vi "InitLinkButtons.vi"(4 "Separator":refnum<vi>, 5 "rightColumnAlignment":refnum<vi>, 6 "Col1Sec3_Top":refnum<vi>, 7 "leftColumnAlignment":refnum<vi>, 8 "icon array":refnum<vi>[](array[refnum]), 9 "button array":refnum<vi>[][](array[refnum]), 10 "Num MRU Items":u16=10, 11 "Pnl Refnum":refnum<vi>) -> (0 "Mode XML Elements":string, 1 "ring info":refnum<class "RingItem.lvclass">[](array[class]), 3 "Handler info":variant)   [LabVIEW 2023, in "GettingStartedWindow.lvlib"]
uses:
  <resource>/modes/FRC/GSW/GettingStartedWindow.lvlib
  <resource>/modes/FRC/GSW/Classes/RingItem/RingItem.lvclass
  <resource>/modes/FRC/GSW/Classes/ClickableText/ClickableText.lvclass
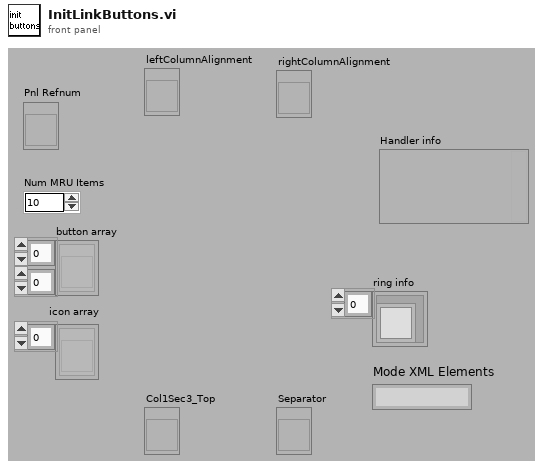
[diagram p1: front panel]
types:
  T1 = cluster{refnum<class "ClickableText.lvclass">[]}[][]
  T2 = typedef "GettingStartedWindow.lvlib/ItemData_Type.ctl" = enum16{"None", "Folder", "New Project", "New VI", "Find", "VI", "Project", "New from template", "RT Project Wizard", "PDA Project Wizard", "Control", "Library", "Class", "XControl", "Runtime menu", "Statechart", "Ladder", "Find LabVIEW Addons", "Instrument Finder", "Example Finder"}
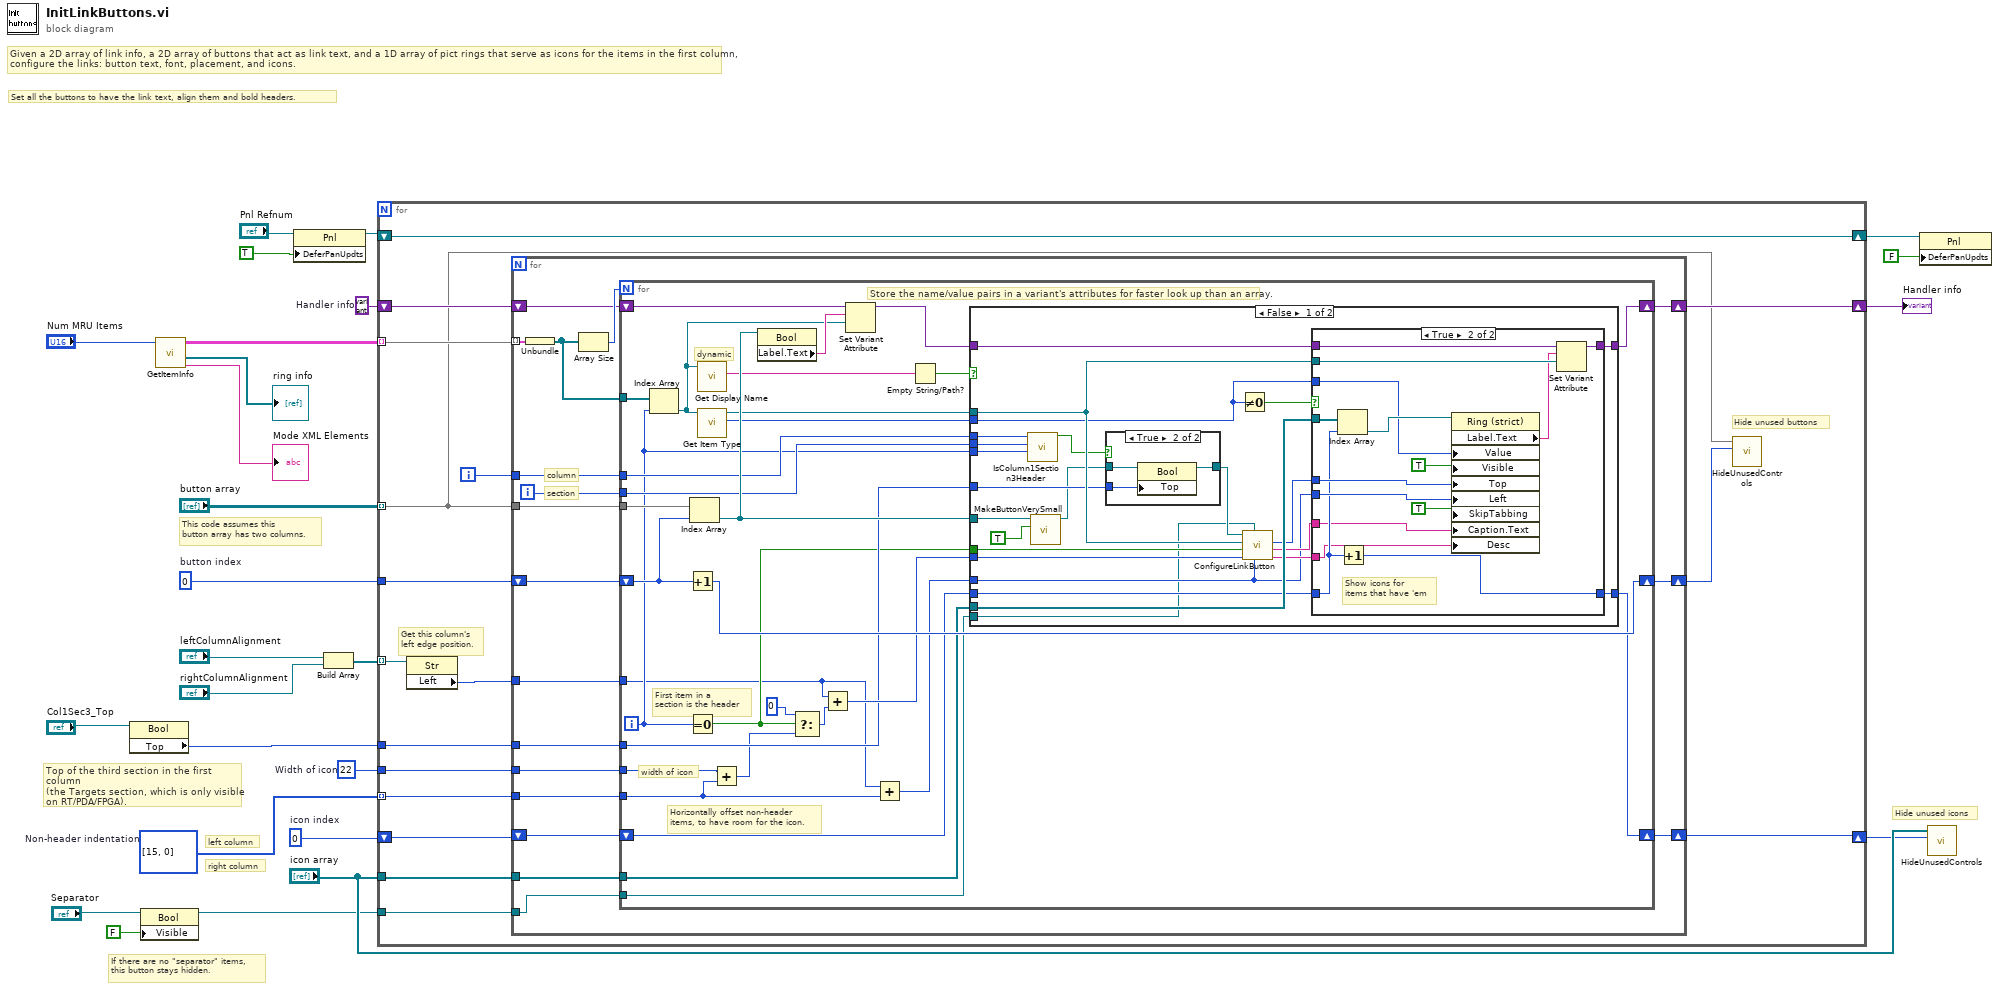
[diagram p0: block diagram]
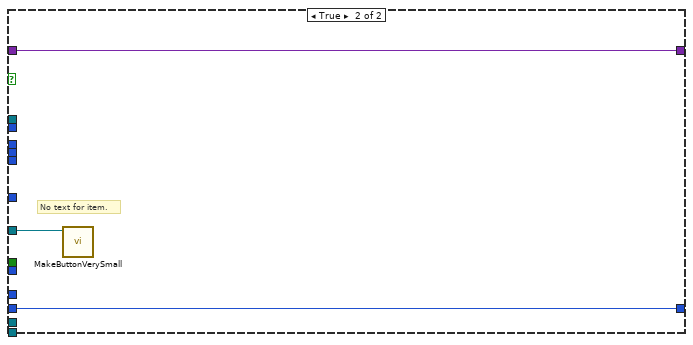
[diagram p4: hidden frame]
diagram:
  w5 = i32[] [15, 0]  # Non-header indentation
  w6 = 0  # button index
  w8 = variant  # Handler info
  w15 = 22  # Width of icon
  w19 = 0  # icon index
  # "If there are no \"separator\" items,\nthis button stays hidden."
  # "right column"
  # "left column"
  # "Set all the buttons to have the link text, align them and bold headers."
  # "Top of the third section in the first column\n(the Targets section, which is only visible\non RT/PDA/FPGA)."
  # "Given a 2D array of link info, a 2D array of buttons that act as link text, and a 1D array of pict rings that serve as icons for the items in the first column,\nconfigure the links: button text, font, placement, and icons."
  # "This code assumes this\nbutton array has two columns."
  # "Hide unused icons"
  n1 = property on="Property Node" class="Bool"(reference="Col1Sec3_Top") -> ("Top"=w12:i32)  [unwired: 1 in, 2 out]
  n2 = property class="Bool"(reference="Separator", "Visible"=FALSE) -> (reference out=w2:refnum<vi>)  [unwired: 1 in, 1 out]
  n3 = call <resource>:"GetItemInfo.vi"("Num MRU Items"="Num MRU Items") -> ("Mode XML Elements"=→"Mode XML Elements":string, "ring info"=→"ring info":refnum<class "RingItem.lvclass">[], "item info array"=w25:T1)  [unwired: 1 in, 7 out]
  n4 = property on="Property Node" class="Pnl"(reference="Pnl Refnum", "DeferPanUpdts"=TRUE ("Defer Panel Updates")) -> (reference out=w22:refnum<vi>)  [unwired: 1 in, 1 out]
  n5 = Build Array("leftColumnAlignment", "rightColumnAlignment") -> (w16:refnum<vi>[])
  n6 = for {
    tunnel: "button array" -> [w31] mode=indexing
    tunnel: w25 -> [w42] mode=indexing
    tunnel: "icon array" -> [w41]
    shift-right: [w39] -> w7
    shift-left: w8 -> [w40]
    shift-right: [w38] -> w20
    shift-left: w22 -> [w38]
    tunnel: w15 -> [w37]
    shift-right: [w35] -> w10
    shift-left: w19 -> [w36]
    tunnel: w16 -> [w34] mode=indexing
    tunnel: w12 -> [w33]
    tunnel: w6 -> [w29]
    tunnel: w5 -> [w28] mode=indexing
    tunnel: w2 -> [w27]
    i -> [w32]
    # "Get this column's\nleft edge position."
    # "Hide unused buttons"
    n7 = property on="Property Node" class="Str"(reference=w34) -> ("Left"=w43:i32)  [unwired: 1 in, 2 out]
    n8 = for {
      tunnel: w31 -> [w61]
      tunnel: w42 -> [w50] mode=indexing
      shift-right: [w59] -> w30
      shift-left: w29 -> [w60]
      tunnel: w43 -> [w58]
      shift-right: [w46] -> w39
      shift-left: w40 -> [w47]
      shift-right: [w56] -> w35
      shift-left: w36 -> [w57]
      tunnel: w41 -> [w55]
      tunnel: w37 -> [w54]
      tunnel: w33 -> [w53]
      tunnel: w32 -> [w52]
      tunnel: w28 -> [w45]
      tunnel: w27 -> [w44]
      i -> [w51]
      # "section"
      # "column"
      n9 = Unbundle(w50) -> (w48:refnum<class "ClickableText.lvclass">[])
      n10 = Array Size(array=w48) -> (size(s)=w49:i32)
      n11 = for {
        N: w49 -> [_]
        tunnel: w48 -> [w86]
        tunnel: w61 -> [w92]
        shift-right: [w90] -> w59
        shift-left: w60 -> [w91]
        tunnel: w58 -> [w65]
        shift-right: [w83] -> w56
        shift-left: w57 -> [w84]
        tunnel: w55 -> [w73]
        tunnel: w54 -> [w67]
        tunnel: w53 -> [w82]
        tunnel: w52 -> [w81]
        tunnel: w51 -> [w80]
        shift-right: [w69] -> w46
        shift-left: w47 -> [w74]
        tunnel: w45 -> [w64]
        tunnel: w44 -> [w62]
        i -> [w79]
        # "dynamic"
        # "First item in a\nsection is the header"
        # "Store the name/value pairs in a variant's attributes for faster look up than an array."
        # "width of icon"
        # "Horizontally offset non-header\nitems, to have room for the icon."
        n12 = Index Array(array=w86, index=w79) -> (element=w75:refnum<class "ClickableText.lvclass">)
        n13 = Increment(x=w91) -> (x+1=w90:i32)
        n14 = Equal To 0?(x=w79) -> (x = 0?=w68:bool)
        n15 = Index Array(array=w92, index=w91) -> (element=w85:refnum<vi>)
        n16 = call-dynamic "Get Display Name.vi"("ClickableText in"=w75) -> ("localized name"=w78:string)  [unwired: 1 in, 9 out]
        n17 = call <resource>:"Get Item Type.vi"("ClickableText in"=w75) -> ("DNL_Type"=w77:T2, "ClickableText out"=w71:refnum<class "ClickableText.lvclass">)  [unwired: 1 in, 8 out]
        n18 = Add(x=w67, y=w64) -> (x+y=w66:i32)
        n19 = property on="Property Node" class="Bool"(reference=w85) -> ("Label.Text"=w76:string)  [unwired: 1 in, 2 out]
        n20 = Select(t=0, s=w68, f=w66) -> (s? t:f=w72:i32)
        n21 = Add(x=w65, y=w72) -> (x+y=w89:i32)
        n22 = Set Variant Attribute(Variant=w74, name=w76, value=w75) -> (Variant out=w70:variant)  [unwired: 1 in, 2 out]
        n23 = Add(x=w65, y=w64) -> (x+y=w63:i32)
        n24 = Empty String/Path?(string/path=w78) -> (empty?=w87:bool)
        n25 = case shown="False" w87 {
          tunnel: w89 -> [w99 _]
          tunnel: w85 -> [w108 w139]
          tunnel: w68 -> [w101 _]
          tunnel: w73 -> [w115 _]
          tunnel: w77 -> [w114 _]
          tunnel: w84 -> [w112 w140]
          tunnel: [w111 w140] -> w83
          tunnel: w63 -> [w94 _]
          tunnel: w82 -> [w110 _]
          tunnel: w81 -> [w105 _]
          tunnel: w80 -> [w104 _]
          tunnel: w79 -> [w103 _]
          tunnel: w71 -> [w116 _]
          tunnel: w70 -> [w98 w138]
          tunnel: [w97 w138] -> w69
          tunnel: w62 -> [w93 _]
          frame False {
            n26 = call <resource>:"IsColumn1Section3Header.vi"("index 3"=w103, "index 2"=w104, "index 1"=w105) -> ("is col 1 section 3 header?"=w106:bool)  [unwired: 1 in, 7 out]
            n27 = call <resource>:"MakeButtonVerySmall.vi"("visible"=TRUE ("Visible"), "Link Button 1"=w108) -> ("Link Button 2"=w107:refnum<vi>)  [unwired: 1 in, 8 out]
            n28 = case shown="True" w106 {
              tunnel: w107 -> [w117 w120]
              tunnel: [w117 w119] -> w102
              tunnel: w110 -> [_ w118]
              frame False {
              }
              frame True {
                n29 = property on="Property Node" class="Bool"(reference=w120, "Top"=w118) -> (reference out=w119:refnum<vi>)  [unwired: 1 in, 1 out]
              }
            }
            n30 = Not Equal To 0?(x=w114) -> (x != 0?=w113:bool)
            n31 = call <resource>:"ConfigureLinkButton.vi"("separator position left"=w94, "Separator"=w93, "Position:Left"=w99, "is section header?"=w101, "GettingStartedWindow.lvlib:ClickableText.lvclass"=w116, "Link Button 1"=w102) -> ("description"=w95:string, "localized name"=w96:string, "Top"=w100:i32)  [unwired: 3 out]
            n32 = case shown="True" w113 {
              tunnel: w114 -> [_ w129]
              tunnel: w115 -> [_ w132]
              tunnel: w112 -> [w122 w130]
              tunnel: [w122 w136] -> w111
              tunnel: w100 -> [_ w135]
              tunnel: w94 -> [_ w134]
              tunnel: w98 -> [w121 w128]
              tunnel: w116 -> [_ w127]
              tunnel: [w121 w126] -> w97
              tunnel: w96 -> [_ w123]
              tunnel: w95 -> [_ w125]
              frame False {
              }
              frame True {
                # "Show icons for\nitems that have 'em"
                n33 = Index Array(array=w132, index=w130) -> (element=w131:refnum<vi>)
                n34 = Increment(x=w130) -> (x+1=w136:i32)
                n35 = property on="Property Node" class="Ring (strict)"(reference=w131, "Value"=w129, "Visible"=TRUE, "Top"=w135, "Left"=w134, "SkipTabbing"=TRUE ("Skip When Tabbing"), "Caption.Text"=w123, "Desc"=w125) -> ("Label.Text"=w124:string)  [unwired: 1 in, 2 out]
                n36 = Set Variant Attribute(Variant=w128, name=w124, value=w127) -> (Variant out=w126:variant)  [unwired: 1 in, 2 out]
              }
            }
          }
          frame True {
            # "No text for item."
            n37 = call <resource>:"MakeButtonVerySmall.vi"("Link Button 1"=w139) -> ()  [unwired: 2 in, 9 out]
          }
        }
      }
    }
    n38 = call <resource>:"HideUnusedControls.vi"("last used index"=w30, "control array"=w31) -> ()  [unwired: 10 out]
  }
  "Handler info" <- w7
  n39 = property on="Property Node" class="Pnl"(reference=w20, "DeferPanUpdts"=FALSE ("Defer Panel Updates")) -> ()  [unwired: 1 in, 2 out]
  n40 = call <resource>:"HideUnusedControls.vi"("last used index"=w10, "control array"="icon array") -> ()  [unwired: 10 out]
